vi "Add Completions Capability.vi"(8 "error in":errorcluster, 11 "result json":string) -> (0 "error out":errorcluster, 3 "result json out":string)   [LabVIEW 2020, in "MCP Server.lvlib"]
doc: "Declares the completions capability (MCP utility completion, answered by completion complete.vi): puts \"completions\":{} first into the capabilities object of the initialize result. result json is the result object as initialize.vi builds it (compact JSON, with a \"capabilities\":{ member); it is returned unchanged when it has none. Used by initialize.vi, so that server/discover, which reads its capabilities from initialize.vi (Read Server Info.vi), declares it too.\n\nRuns regardless of error in, which is passed through unchanged."
uses:
  MCP Server.lvlib
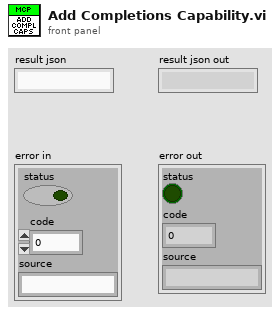
[diagram p1: front panel]
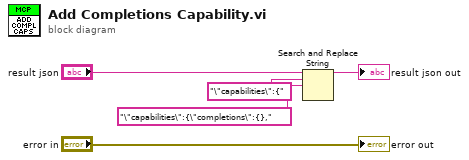
[diagram p0: block diagram]
diagram:
  n1 = Search and Replace String(input string="result json", search string="\"capabilities\":{" ("capabilities"), replace string="\"capabilities\":{\"completions\":{}," ("with completions")) -> (result string=→"result json out":string)  [unwired: 5 in, 3 out]
  "error out" <- "error in"
